vi "Release.vi"(8 "error in (no error)":errorcluster, 11 "Execution in":refnum<class "Execution.lvclass">) -> (0 "error out":errorcluster)   [LabVIEW 2020, in "TSnax.lvlib" / "Execution.lvclass"]
uses:
  Execution.lvclass
  Execution.lvclass/Execution.ctl
  PropertyObject/PropertyObject.lvclass/PropertyObject.ctl
  PropertyObject/PropertyObject Ref.vi
  SequenceFile/SequenceFile.lvclass
  C:/dev/illuminated-g/tsnax/TSnax/PropertyObject/PropertyObject.lvclass
  PropertyObject/PropertyObject.lvclass
  C:/dev/illuminated-g/tsnax/TSnax/PropertyObjectFile/PropertyObjectFile.lvclass
  C:/dev/illuminated-g/tsnax/TSnax/SequenceFile/SequenceFile.lvclass
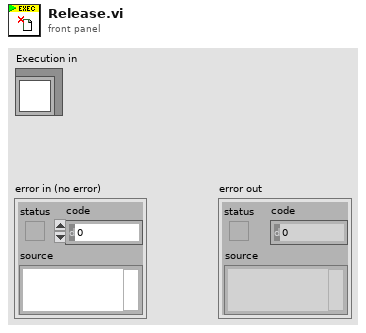
[diagram p1: front panel]
types:
  T1 = typedef "TSnax.lvlib/Execution.lvclass/Ref Data.ctl" = cluster{"Parameters":refnum<class "PropertyObject.lvclass">, "Client Sequence":refnum<class "SequenceFile.lvclass">, "Process Model":refnum<class "SequenceFile.lvclass">, "Entry Sequence":string, "Execution":refnum<k7>, "Report":refnum<class "Report.lvclass">, "Options":T2, "Started":bool, "Complete":bool, "UIMsg Callback ID":i32}
  T2 = typedef "TSnax.lvlib/Execution Options.ctl" = cluster{"Use Default Model (T)":bool, "Release Related References (T)":bool}
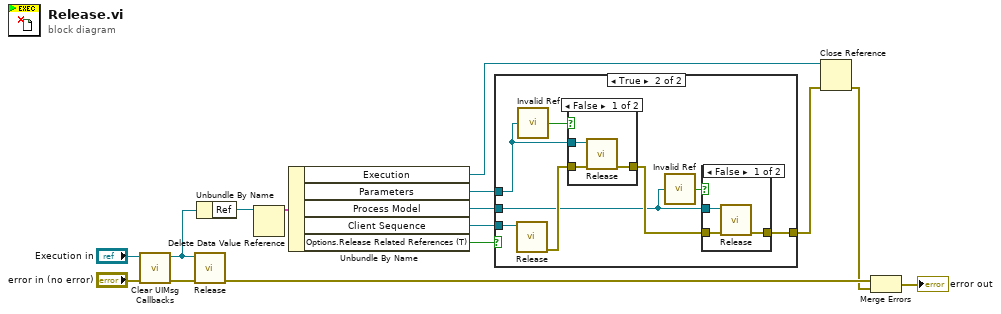
[diagram p0: block diagram]
diagram:
  n1 = call "Clear UIMsg Callbacks.vi"("error in (no error)"="error in (no error)", "Execution in"="Execution in") -> ("error out"=w1:errorcluster, "Execution out"=w2:refnum<class "Execution.lvclass">)  [unwired: 8 in]
  n2 = call-parent "Release.vi"("error in (no error)"=w1, "PropertyObject in"=w2) -> ("error out"=w7:errorcluster)  [unwired: 9 in]
  n3 = Unbundle By Name(w2) -> ("Ref"=w15:refnum<data-value>)
  n4 = Delete Data Value Reference(data value reference=w15) -> (data value=w14:T1)  [unwired: 1 in, 1 out]
  n5 = Unbundle By Name(w14) -> ("Execution"=w9:refnum<k7>, "Parameters"=w10:refnum<class "PropertyObject.lvclass">, "Process Model"=w11:refnum<class "SequenceFile.lvclass">, "Client Sequence"=w12:refnum<class "SequenceFile.lvclass">, "Options.Release Related References (T)"=w13:bool)
  n6 = case shown="True" w13 {
    tunnel: w12 -> [_ w23]
    tunnel: w11 -> [_ w17]
    tunnel: w10 -> [_ w21]
    tunnel: [_ w16] -> w8
    frame False {
    }
    frame True {
      n7 = call-dynamic "Release.vi"("SequenceFile in"=w23) -> ("error out"=w20:errorcluster)  [unwired: 10 in]
      n8 = call "Invalid Ref.vi"("PropertyObject"=w21) -> ("Not a Valid Ref?"=w22:bool)
      n9 = case shown="False" w22 {
        tunnel: w21 -> [w30 _]
        tunnel: [w29 w31] -> w18
        tunnel: w20 -> [w28 w31]
        frame False {
          n10 = call-dynamic "Release.vi"("error in (no error)"=w28, "PropertyObject in"=w30) -> ("error out"=w29:errorcluster)  [unwired: 9 in]
        }
        frame True {
        }
      }
      n11 = call "Invalid Ref.vi"("PropertyObject"=w17) -> ("Not a Valid Ref?"=w19:bool)
      n12 = case shown="False" w19 {
        tunnel: w17 -> [w26 _]
        tunnel: [w25 w27] -> w16
        tunnel: w18 -> [w24 w27]
        frame False {
          n13 = call-dynamic "Release.vi"("error in (no error)"=w24, "SequenceFile in"=w26) -> ("error out"=w25:errorcluster)  [unwired: 9 in]
        }
        frame True {
        }
      }
    }
  }
  n14 = Close Reference(reference=w9, error in (no error)=w8) -> (error out=w6:errorcluster)
  n15 = Merge Errors(w7, w6) -> (→"error out":errorcluster)
